vi "W_ID_arr.vi"(8 "error in (no error)":errorcluster caption="错误输入（无错误）", 10 "ID_arr":string[](array[string]), 11 "Procotol_class输入":refnum<class "Procotol_class.lvclass">) -> (0 "error out":errorcluster caption="错误输出", 3 "Procotol_class输出":refnum<class "Procotol_class.lvclass">)   [LabVIEW 2025, in "Procotol_class.lvclass"]
uses:
  Procotol_class.lvclass
  Procotol_class.lvclass/Procotol_class.ctl
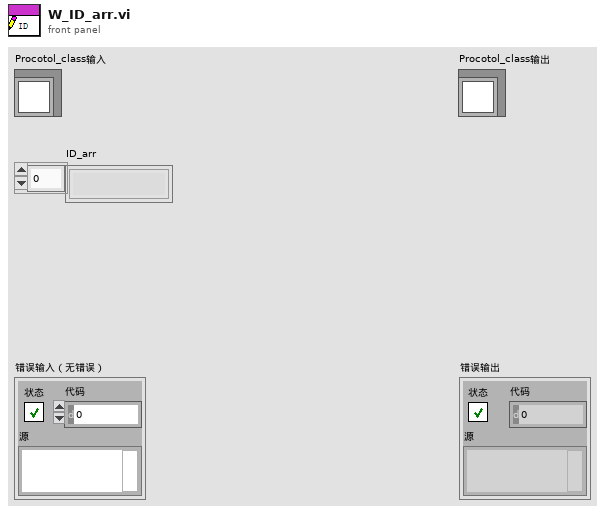
[diagram p1: front panel]
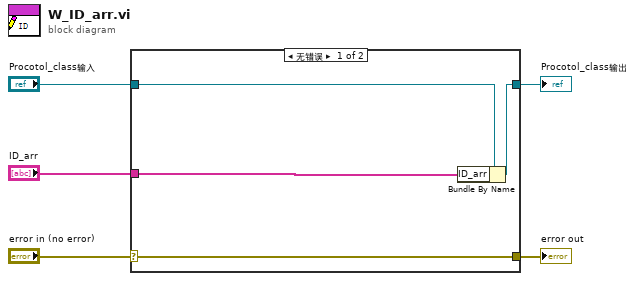
[diagram p0: block diagram]
diagram:
  n1 = case shown="无错误" "error in (no error)" {
    selector: "error in (no error)" -> [w9 w10]
    tunnel: [w9 w10] -> w4
    tunnel: [w7 w11] -> w2
    tunnel: "Procotol_class输入" -> [w8 w11]
    tunnel: "ID_arr" -> [w6 _]
    frame No Error {
      n2 = Bundle By Name(cluster=w8, "ID_arr"=w6) -> (w7:refnum<class "Procotol_class.lvclass">)
    }
    frame Error {
    }
  }
  "error out" <- w4
  "Procotol_class输出" <- w2
